vi "JKI SM Editor - VIPC File -- List Packages__vipm_api_vipm_api.vi"(8 "error in (no error)":errorcluster, 11 "VIPC File Path":path) -> (0 "error out":errorcluster, 1 "VIPC LabVIEW Version":string, 2 "Package List":string[](array[string]), 3 "VIPC File Path (dup)":path)   [LabVIEW 2020]
doc: "Copyright 2009-2012 JKI"
uses:
  <userlib>/_OpenG.lib/lvzip/lvzip.llb/subVI/ZLIB Open Unzip Archive (Path)__ogtk.vi
  <userlib>/_OpenG.lib/lvzip/lvzip.llb/ZLIB Extract Stream__ogtk.vi
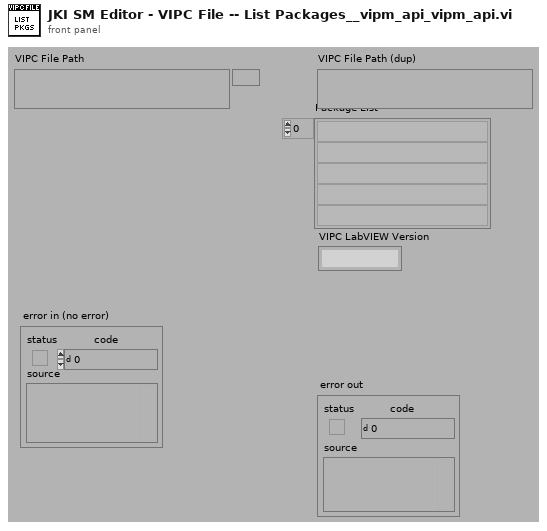
[diagram p1: front panel]
types:
  T1 = typedef "ZLIB Unzip Handle__ogtk.ctl" = refnum<k1>
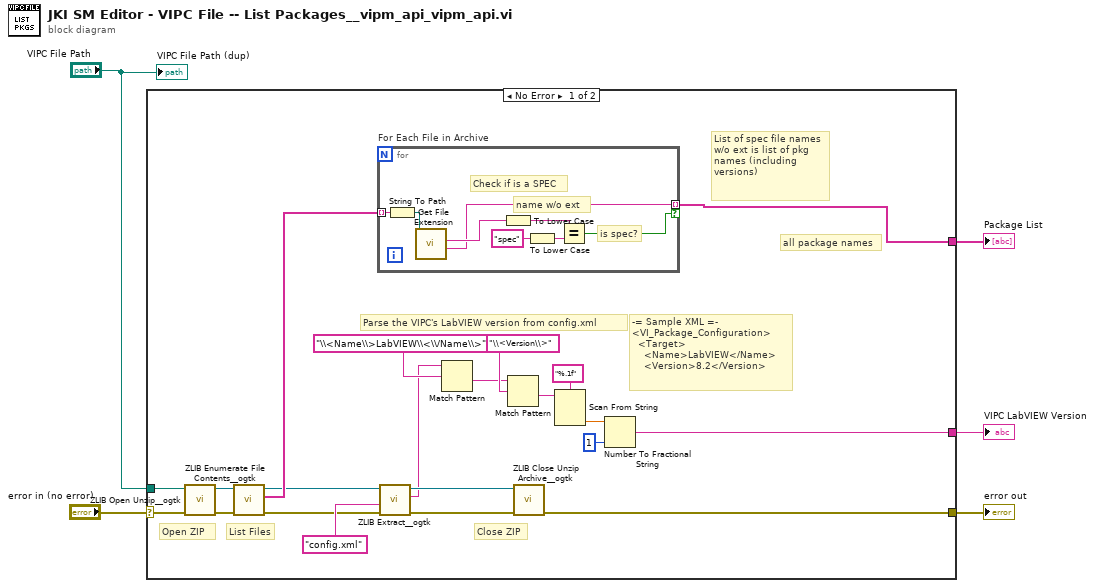
[diagram p0: block diagram]
diagram:
  n1 = case shown="No Error" "error in (no error)" {
    selector: "error in (no error)" -> [w8 w35]
    tunnel: [w6 _] -> w4
    tunnel: [w7 w35] -> w3
    tunnel: "VIPC File Path" -> [w18 _]
    tunnel: [w19 _] -> w1
    frame No Error {
      # "all package names"
      # "-= Sample XML =-\n<VI_Package_Configuration>\n  <Target>\n    <Name>LabVIEW</Name>\n    <Version>8.2</Version>"
      # "Parse the VIPC's LabVIEW version from config.xml"
      # "Close ZIP"
      # "List Files"
      # "Open ZIP"
      # "List of spec file names w/o ext is list of pkg names (including versions)"
      n2 = call-poly <userlib>:"ZLIB Open Unzip__ogtk.vi"("error in (no error)"=w8, "archive name"=w18) -> ("error out"=w9:errorcluster, "unzip Refnum"=w17:T1)  [unwired: 4 in]
      n3 = call <userlib>:"ZLIB Enumerate File Contents__ogtk.vi"("error in (no error)"=w9, "unzip Refnum"=w17) -> ("error out"=w10:errorcluster, "file names"=w16:string[], "unzip Refnum out"=w14:T1)  [unwired: 5 in, 2 out]
      n4 = for "For Each File in Archive" {
        tunnel: w16 -> [w31] mode=indexing
        tunnel: [w29] -> w6 mode=indexing if=w27
        # "is spec?"
        # "name w/o ext"
        # "Check if is a SPEC"
        n5 = String To Path(string=w31) -> (path=w28:path)
        n6 = call <vilib>:"Get File Extension.vi"("file"=w28) -> ("filename without extension"=w29:string, "lowercase file extension"=w30:string)  [unwired: 6 in, 3 out]
        n7 = To Lower Case(string=w30) -> (all lower case string=w33:string)
        n8 = To Lower Case(string="spec" ("extension")) -> (all lower case string=w32:string)
        n9 = Equal?(x=w33, y=w32) -> (x = y?=w27:bool)
      }
      n10 = call-poly <userlib>:"ZLIB Extract__ogtk.vi"("error in (no error)"=w10, "internal name"="config.xml" ("extension"), "unzip Refnum"=w14) -> ("error out"=w11:errorcluster, "byte stream"=w12:string, "unzip Refnum out"=w13:T1)  [unwired: 3 in, 1 out]
      n11 = Match Pattern(string=w12, regular expression="\\<Name\\>LabVIEW\\<\\/Name\\>") -> (after substring=w24:string)  [unwired: 1 in, 3 out]
      n12 = Match Pattern(string=w24, regular expression="\\<Version\\>") -> (after substring=w21:string)  [unwired: 1 in, 3 out]
      n13 = call <userlib>:"ZLIB Close Unzip Archive__ogtk.vi"("error in (no error)"=w11, "unzip Refnum"=w13) -> ("error out"=w7:errorcluster)  [unwired: 4 in, 1 out]
      n14 = Scan From String(format string="%.1f", input string=w21) -> (output 1=w22:dbl)  [unwired: 3 in, 3 out]
      n15 = Number To Fractional String(number=w22, precision (6)=i16 1) -> (F-format string=w19:string)  [unwired: 2 in]
    }
    frame Error {
    }
  }
  "error out" <- w3
  "Package List" <- w4
  "VIPC LabVIEW Version" <- w1
  "VIPC File Path (dup)" <- "VIPC File Path"
